vi "Global_SKM.vi"() -> ()   [LabVIEW 2025]
uses:
  Working condition setting_SKM.ctl
  data structure.ctl
panel:
  out "Stop":bool
  out "Wet Temp/RH":string[](array[string])
  in  "Information":string[][](array[string])=[["Date & Time", "02/23/2023 15:53:17"], ["Equipment Type Tested", "Chiller"], ["Refrigerant Type", ""], ["Operator Name", "qwe"], ["Test Duration (Time started/finished)", "fgh"], ["Job Reference Number", "120-20230209-01"], ["Unit Serial Number/EPN/SO Number", ""], ["Power Supply", ""], ["IPLV", ""], ["Test Report Number", ""], ["Refrigerant Charge", ""], ["Manufacturer/Brand Name", ""], ["Model Name/Series", ""], ["Test Standard", ""], ["Evaporator Type", ""], ["Evaporator Configuration", ""], ["Qty of Evaporator", ""], ["Evaporator 1 Model", ""], ["Evaporator 2 Model", ""], ["Evaporator 1 Serial #", ""], ["Evaporator 2 Serial #", ""], ["Condenser Type", ""], ["Qty of Condenser", ""], ["Number of Fans", ""], ["Number of actual running fans", ""], ["Rated Fan Speed", ""], ["Average Actual Fan Speed", ""], ["Rated Fan Motor Ampere", ""], ["Average Actual Fan Motor Ampere", ""], ["Qty of Compressor/Ckt", ""], ["Compressor Type", ""], ["Compressor Model", ""], ["Compressor Serial Number", ""], ["Refrigerant Charge", ""], ["Compressor Rated Load Amps", ""], ["Compressor Actual Ampere Drawn", ""], ["Compressor Type_Ckt2", ""], ["Compressor Model_Ckt2", ""], ["Compressor Serial Number_Ckt2", ""], ["Refrigerant Charge_Ckt2", ""], ["Compressor Rated Load Amps_Ckt2", ""], ["Compressor Actual Ampere Drawn_Ckt2", ""], ["Compressor Type_Ckt3", ""], ["Compressor Model_Ckt3", ""], ["Compressor Serial Number_Ckt3", ""], ["Refrigerant Charge_Ckt3", ""], ["Compressor Rated Load Amps_Ckt3", ""], ["Compressor Actual Ampere Drawn_Ckt3", ""], ["Compressor Type_Ckt4", ""], ["Compressor Model_Ckt4", ""], ["Compressor Serial Number_Ckt4", ""], ["Refrigerant Charge_Ckt4", ""], ["Compressor Rated Load Amps_Ckt4", ""], ["Compressor Actual Ampere Drawn_Ckt4", ""], ["Compressor Type_Ckt5", ""], ["Compressor Model_Ckt5", ""], ["Compressor Serial Number_Ckt5", ""], ["Refrigerant Charge_Ckt5", ""], ["Compressor Rated Load Amps_Ckt5", ""], ["Compressor Actual Ampere Drawn_Ckt5", ""], ["Compressor Type_Ckt6", ""], ["Compressor Model_Ckt6", ""], ["Compressor Serial Number_Ckt6", ""], ["Refrigerant Charge_Ckt6", ""], ["Compressor Rated Load Amps_Ckt6", ""], ["Compressor Actual Ampere Drawn_Ckt6", ""], ["Compressor Type_Ckt7", ""], ["Compressor Model_Ckt7", ""], ["Compressor Serial Number_Ckt7", ""], ["Refrigerant Charge_Ckt7", ""], ["Compressor Rated Load Amps_Ckt7", ""], ["Compressor Actual Ampere Drawn_Ckt7", ""], ["Compressor Type_Ckt8", ""], ["Compressor Model_Ckt8", ""], ["Compressor Serial Number_Ckt8", ""], ["Refrigerant Charge_Ckt8", ""], ["Compressor Rated Load Amps_Ckt8", ""], ["Compressor Actual Ampere Drawn_Ckt8", ""], ["Exp Valve Opening_Ckt1 ", ""], ["Exp Valve Opening_Ckt2", ""], ["Exp Valve Opening_Ckt3", ""], ["Exp Valve Opening_Ckt4", ""], ["Exp Valve Opening_Ckt5", ""], ["Exp Valve Opening_Ckt6", ""], ["Exp Valve Opening_Ckt7", ""], ["Exp Valve Opening_Ckt8", ""]]
  out "simu":bool
  in  "Correction_Data":dbl[][][](array[numeric])
  in  "数据结构组":T1[](array[typedef])=[{"展示名称"="U1_1", "单位"="V", "值"="", "物理通道"=240, "逻辑通道"=0, "小数点"=2, "数值"=0.0, "修正因子"={"a"=0.0, "b"=1.0, "c"=0.0}, "原始值"=0.0, "逻辑名称"="U1_1"}, {"展示名称"="I1_1", "单位"="A", "值"="", "物理通道"=241, "逻辑通道"=1, "小数点"=2, "数值"=0.0, "修正因子"={"a"=0.0, "b"=1.0, "c"=0.0}, "原始值"=0.0, "逻辑名称"="I1_1"}, {"展示名称"="P1_1", "单位"="W", "值"="", "物理通道"=242, "逻辑通道"=2, "小数点"=2, "数值"=0.0, "修正因子"={"a"=0.0, "b"=1.0, "c"=0.0}, "原始值"=0.0, "逻辑名称"="P1_1"}, {"展示名称"="E1_1", "单位"="W·h", "值"="", "物理通道"=243, "逻辑通道"=3, "小数点"=2, "数值"=0.0, "修正因子"={"a"=0.0, "b"=1.0, "c"=0.0}, "原始值"=0.0, "逻辑名称"="E1_1"}, {"展示名称"="U1_2", "单位"="V", "值"="", "物理通道"=244, "逻辑通道"=4, "小数点"=2, "数值"=0.0, "修正因子"={"a"=0.0, "b"=1.0, "c"=0.0}, "原始值"=0.0, "逻辑名称"="U1_2"}, {"展示名称"="I1_2", "单位"="A", "值"="", "物理通道"=245, "逻辑通道"=5, "小数点"=2, "数值"=0.0, "修正因子"={"a"=0.0, "b"=1.0, "c"=0.0}, "原始值"=0.0, "逻辑名称"="I1_2"}, {"展示名称"="P1_2", "单位"="W", "值"="", "物理通道"=246, "逻辑通道"=6, "小数点"=2, "数值"=0.0, "修正因子"={"a"=0.0, "b"=1.0, "c"=0.0}, "原始值"=0.0, "逻辑名称"="P1_2"}, {"展示名称"="E1_2", "单位"="W·h", "值"="", "物理通道"=247, "逻辑通道"=7, "小数点"=2, "数值"=0.0, "修正因子"={"a"=0.0, "b"=1.0, "c"=0.0}, "原始值"=0.0, "逻辑名称"="E1_2"}, {"展示名称"="U1_3", "单位"="V", "值"="", "物理通道"=248, "逻辑通道"=8, "小数点"=2, "数值"=0.0, "修正因子"={"a"=0.0, "b"=1.0, "c"=0.0}, "原始值"=0.0, "逻辑名称"="U1_3"}, {"展示名称"="I1_3", "单位"="A", "值"="", "物理通道"=249, "逻辑通道"=9, "小数点"=2, "数值"=0.0, "修正因子"={"a"=0.0, "b"=1.0, "c"=0.0}, "原始值"=0.0, "逻辑名称"="I1_3"}, {"展示名称"="P1_3", "单位"="W", "值"="", "物理通道"=250, "逻辑通道"=10, "小数点"=2, "数值"=0.0, "修正因子"={"a"=0.0, "b"=1.0, "c"=0.0}, "原始值"=0.0, "逻辑名称"="P1_3"}, {"展示名称"="E1_3", "单位"="W·h", "值"="", "物理通道"=251, "逻辑通道"=11, "小数点"=2, "数值"=0.0, "修正因子"={"a"=0.0, "b"=1.0, "c"=0.0}, "原始值"=0.0, "逻辑名称"="E1_3"}, {"展示名称"="U1_4", "单位"="V", "值"="", "物理通道"=252, "逻辑通道"=12, "小数点"=2, "数值"=0.0, "修正因子"={"a"=0.0, "b"=1.0, "c"=0.0}, "原始值"=0.0, "逻辑名称"="U1_4"}, {"展示名称"="I1_4", "单位"="A", "值"="", "物理通道"=253, "逻辑通道"=13, "小数点"=2, "数值"=0.0, "修正因子"={"a"=0.0, "b"=1.0, "c"=0.0}, "原始值"=0.0, "逻辑名称"="I1_4"}, {"展示名称"="P1_4", "单位"="W", "值"="", "物理通道"=254, "逻辑通道"=14, "小数点"=3, "数值"=0.0, "修正因子"={"a"=0.0, "b"=1.0, "c"=0.0}, "原始值"=0.0, "逻辑名称"="P1_4"}, {"展示名称"="E1_4", "单位"="W·h", "值"="", "物理通道"=255, "逻辑通道"=15, "小数点"=3, "数值"=0.0, "修正因子"={"a"=0.0, "b"=1.0, "c"=0.0}, "原始值"=0.0, "逻辑名称"="E1_4"}, {"展示名称"="Fq1", "单位"="Hz", "值"="", "物理通道"=256, "逻辑通道"=16, "小数点"=3, "数值"=0.0, "修正因子"={"a"=0.0, "b"=1.0, "c"=0.0}, "原始值"=0.0, "逻辑名称"="Fq1"}, {"展示名称"="Factor1", "单位"="", "值"="", "物理通道"=257, "逻辑通道"=17, "小数点"=3, "数值"=0.0, "修正因子"={"a"=0.0, "b"=1.0, "c"=0.0}, "原始值"=0.0, "逻辑名称"="Factor1"}, {"展示名称"="U2_1", "单位"="V", "值"="", "物理通道"=260, "逻辑通道"=18, "小数点"=1, "数值"=0.0, "修正因子"={"a"=0.0, "b"=1.0, "c"=0.0}, "原始值"=0.0, "逻辑名称"="U2_1"}, {"展示名称"="I2_1", "单位"="A", "值"="", "物理通道"=261, "逻辑通道"=19, "小数点"=1, "数值"=0.0, "修正因子"={"a"=0.0, "b"=1.0, "c"=0.0}, "原始值"=0.0, "逻辑名称"="I2_1"}, {"展示名称"="P2_1", "单位"="W", "值"="", "物理通道"=262, "逻辑通道"=20, "小数点"=1, "数值"=0.0, "修正因子"={"a"=0.0, "b"=1.0, "c"=0.0}, "原始值"=0.0, "逻辑名称"="P2_1"}, {"展示名称"="E2_1", "单位"="W·h", "值"="", "物理通道"=263, "逻辑通道"=21, "小数点"=2, "数值"=0.0, "修正因子"={"a"=0.0, "b"=1.0, "c"=0.0}, "原始值"=0.0, "逻辑名称"="E2_1"}, {"展示名称"="U2_2", "单位"="V", "值"="", "物理通道"=264, "逻辑通道"=22, "小数点"=2, "数值"=0.0, "修正因子"={"a"=0.0, "b"=1.0, "c"=0.0}, "原始值"=0.0, "逻辑名称"="U2_2"}, {"展示名称"="I2_2", "单位"="A", "值"="", "物理通道"=265, "逻辑通道"=23, "小数点"=2, "数值"=0.0, "修正因子"={"a"=0.0, "b"=1.0, "c"=0.0}, "原始值"=0.0, "逻辑名称"="I2_2"}, {"展示名称"="P2_2", "单位"="W", "值"="", "物理通道"=266, "逻辑通道"=24, "小数点"=2, "数值"=0.0, "修正因子"={"a"=0.0, "b"=1.0, "c"=0.0}, "原始值"=0.0, "逻辑名称"="P2_2"}, {"展示名称"="E2_2", "单位"="W·h", "值"="", "物理通道"=267, "逻辑通道"=25, "小数点"=1, "数值"=0.0, "修正因子"={"a"=0.0, "b"=1.0, "c"=0.0}, "原始值"=0.0, "逻辑名称"="E2_2"}, {"展示名称"="U2_3", "单位"="V", "值"="", "物理通道"=268, "逻辑通道"=26, "小数点"=1, "数值"=0.0, "修正因子"={"a"=0.0, "b"=1.0, "c"=0.0}, "原始值"=0.0, "逻辑名称"="U2_3"}, {"展示名称"="I2_3", "单位"="A", "值"="", "物理通道"=269, "逻辑通道"=27, "小数点"=1, "数值"=0.0, "修正因子"={"a"=0.0, "b"=1.0, "c"=0.0}, "原始值"=0.0, "逻辑名称"="I2_3"}, {"展示名称"="P2_3", "单位"="W", "值"="", "物理通道"=270, "逻辑通道"=28, "小数点"=1, "数值"=0.0, "修正因子"={"a"=0.0, "b"=1.0, "c"=0.0}, "原始值"=0.0, "逻辑名称"="P2_3"}, {"展示名称"="E2_3", "单位"="W·h", "值"="", "物理通道"=271, "逻辑通道"=29, "小数点"=1, "数值"=0.0, "修正因子"={"a"=0.0, "b"=1.0, "c"=0.0}, "原始值"=0.0, "逻辑名称"="E2_3"}, {"展示名称"="U2_4", "单位"="V", "值"="", "物理通道"=272, "逻辑通道"=30, "小数点"=1, "数值"=0.0, "修正因子"={"a"=0.0, "b"=1.0, "c"=0.0}, "原始值"=0.0, "逻辑名称"="U2_4"}, {"展示名称"="I2_4", "单位"="A", "值"="", "物理通道"=273, "逻辑通道"=31, "小数点"=1, "数值"=0.0, "修正因子"={"a"=0.0, "b"=1.0, "c"=0.0}, "原始值"=0.0, "逻辑名称"="I2_4"}, {"展示名称"="P2_4", "单位"="W", "值"="", "物理通道"=274, "逻辑通道"=32, "小数点"=1, "数值"=0.0, "修正因子"={"a"=0.0, "b"=1.0, "c"=0.0}, "原始值"=0.0, "逻辑名称"="P2_4"}, {"展示名称"="E2_4", "单位"="W·h", "值"="", "物理通道"=275, "逻辑通道"=33, "小数点"=1, "数值"=0.0, "修正因子"={"a"=0.0, "b"=1.0, "c"=0.0}, "原始值"=0.0, "逻辑名称"="E2_4"}, {"展示名称"="Fq2", "单位"="Hz", "值"="", "物理通道"=276, "逻辑通道"=34, "小数点"=1, "数值"=0.0, "修正因子"={"a"=0.0, "b"=1.0, "c"=0.0}, "原始值"=0.0, "逻辑名称"="Fq2"}, {"展示名称"="Factor2", "单位"="", "值"="", "物理通道"=277, "逻辑通道"=35, "小数点"=1, "数值"=0.0, "修正因子"={"a"=0.0, "b"=1.0, "c"=0.0}, "原始值"=0.0, "逻辑名称"="Factor2"}, {"展示名称"="U3_1", "单位"="V", "值"="", "物理通道"=280, "逻辑通道"=36, "小数点"=1, "数值"=0.0, "修正因子"={"a"=0.0, "b"=1.0, "c"=0.0}, "原始值"=0.0, "逻辑名称"="U3_1"}, {"展示名称"="I3_1", "单位"="A", "值"="", "物理通道"=281, "逻辑通道"=37, "小数点"=1, "数值"=0.0, "修正因子"={"a"=0.0, "b"=1.0, "c"=0.0}, "原始值"=0.0, "逻辑名称"="I3_1"}, {"展示名称"="P3_1", "单位"="W", "值"="", "物理通道"=282, "逻辑通道"=38, "小数点"=1, "数值"=0.0, "修正因子"={"a"=0.0, "b"=1.0, "c"=0.0}, "原始值"=0.0, "逻辑名称"="P3_1"}, {"展示名称"="E3_1", "单位"="W·h", "值"="", "物理通道"=283, "逻辑通道"=39, "小数点"=1, "数值"=0.0, "修正因子"={"a"=0.0, "b"=1.0, "c"=0.0}, "原始值"=0.0, "逻辑名称"="E3_1"}, {"展示名称"="U3_2", "单位"="V", "值"="", "物理通道"=284, "逻辑通道"=40, "小数点"=1, "数值"=0.0, "修正因子"={"a"=0.0, "b"=1.0, "c"=0.0}, "原始值"=0.0, "逻辑名称"="U3_2"}, {"展示名称"="I3_2", "单位"="A", "值"="", "物理通道"=285, "逻辑通道"=41, "小数点"=1, "数值"=0.0, "修正因子"={"a"=0.0, "b"=1.0, "c"=0.0}, "原始值"=0.0, "逻辑名称"="I3_2"}, {"展示名称"="P3_2", "单位"="W", "值"="", "物理通道"=286, "逻辑通道"=42, "小数点"=1, "数值"=0.0, "修正因子"={"a"=0.0, "b"=1.0, "c"=0.0}, "原始值"=0.0, "逻辑名称"="P3_2"}, {"展示名称"="E3_2", "单位"="W·h", "值"="", "物理通道"=287, "逻辑通道"=43, "小数点"=1, "数值"=0.0, "修正因子"={"a"=0.0, "b"=1.0, "c"=0.0}, "原始值"=0.0, "逻辑名称"="E3_2"}, {"展示名称"="U3_3", "单位"="V", "值"="", "物理通道"=288, "逻辑通道"=44, "小数点"=1, "数值"=0.0, "修正因子"={"a"=0.0, "b"=1.0, "c"=0.0}, "原始值"=0.0, "逻辑名称"="U3_3"}, {"展示名称"="I3_3", "单位"="A", "值"="", "物理通道"=289, "逻辑通道"=45, "小数点"=1, "数值"=0.0, "修正因子"={"a"=0.0, "b"=1.0, "c"=0.0}, "原始值"=0.0, "逻辑名称"="I3_3"}, {"展示名称"="P3_3", "单位"="W", "值"="", "物理通道"=290, "逻辑通道"=46, "小数点"=1, "数值"=0.0, "修正因子"={"a"=0.0, "b"=1.0, "c"=0.0}, "原始值"=0.0, "逻辑名称"="P3_3"}, {"展示名称"="E3_3", "单位"="W·h", "值"="", "物理通道"=291, "逻辑通道"=47, "小数点"=1, "数值"=0.0, "修正因子"={"a"=0.0, "b"=1.0, "c"=0.0}, "原始值"=0.0, "逻辑名称"="E3_3"}, {"展示名称"="U3_4", "单位"="V", "值"="", "物理通道"=292, "逻辑通道"=48, "小数点"=1, "数值"=0.0, "修正因子"={"a"=0.0, "b"=1.0, "c"=0.0}, "原始值"=0.0, "逻辑名称"="U3_4"}, {"展示名称"="I3_4", "单位"="A", "值"="", "物理通道"=293, "逻辑通道"=49, "小数点"=1, "数值"=0.0, "修正因子"={"a"=0.0, "b"=1.0, "c"=0.0}, "原始值"=0.0, "逻辑名称"="I3_4"}, {"展示名称"="P3_4", "单位"="W", "值"="", "物理通道"=294, "逻辑通道"=50, "小数点"=1, "数值"=0.0, "修正因子"={"a"=0.0, "b"=1.0, "c"=0.0}, "原始值"=0.0, "逻辑名称"="P3_4"}, {"展示名称"="E3_4", "单位"="W·h", "值"="", "物理通道"=295, "逻辑通道"=51, "小数点"=1, "数值"=0.0, "修正因子"={"a"=0.0, "b"=1.0, "c"=0.0}, "原始值"=0.0, "逻辑名称"="E3_4"}, {"展示名称"="Fq3", "单位"="Hz", "值"="", "物理通道"=296, "逻辑通道"=52, "小数点"=1, "数值"=0.0, "修正因子"={"a"=0.0, "b"=1.0, "c"=0.0}, "原始值"=0.0, "逻辑名称"="Fq3"}, {"展示名称"="Factor3", "单位"="", "值"="", "物理通道"=297, "逻辑通道"=53, "小数点"=1, "数值"=0.0, "修正因子"={"a"=0.0, "b"=1.0, "c"=0.0}, "原始值"=0.0, "逻辑名称"="Factor3"}, {"展示名称"="U4_1", "单位"="V", "值"="", "物理通道"=300, "逻辑通道"=54, "小数点"=1, "数值"=0.0, "修正因子"={"a"=0.0, "b"=1.0, "c"=0.0}, "原始值"=0.0, "逻辑名称"="U4_1"}, {"展示名称"="I4_1", "单位"="A", "值"="", "物理通道"=301, "逻辑通道"=55, "小数点"=1, "数值"=0.0, "修正因子"={"a"=0.0, "b"=1.0, "c"=0.0}, "原始值"=0.0, "逻辑名称"="I4_1"}, {"展示名称"="P4_1", "单位"="W", "值"="", "物理通道"=302, "逻辑通道"=56, "小数点"=1, "数值"=0.0, "修正因子"={"a"=0.0, "b"=1.0, "c"=0.0}, "原始值"=0.0, "逻辑名称"="P4_1"}, {"展示名称"="E4_1", "单位"="W·h", "值"="", "物理通道"=303, "逻辑通道"=57, "小数点"=1, "数值"=0.0, "修正因子"={"a"=0.0, "b"=1.0, "c"=0.0}, "原始值"=0.0, "逻辑名称"="E4_1"}, {"展示名称"="U4_2", "单位"="V", "值"="", "物理通道"=304, "逻辑通道"=58, "小数点"=1, "数值"=0.0, "修正因子"={"a"=0.0, "b"=1.0, "c"=0.0}, "原始值"=0.0, "逻辑名称"="U4_2"}, {"展示名称"="I4_2", "单位"="A", "值"="", "物理通道"=305, "逻辑通道"=59, "小数点"=1, "数值"=0.0, "修正因子"={"a"=0.0, "b"=1.0, "c"=0.0}, "原始值"=0.0, "逻辑名称"="I4_2"}, {"展示名称"="P4_2", "单位"="W", "值"="", "物理通道"=306, "逻辑通道"=60, "小数点"=1, "数值"=0.0, "修正因子"={"a"=0.0, "b"=1.0, "c"=0.0}, "原始值"=0.0, "逻辑名称"="P4_2"}, {"展示名称"="E4_2", "单位"="W·h", "值"="", "物理通道"=307, "逻辑通道"=61, "小数点"=1, "数值"=0.0, "修正因子"={"a"=0.0, "b"=1.0, "c"=0.0}, "原始值"=0.0, "逻辑名称"="E4_2"}, {"展示名称"="U4_3", "单位"="V", "值"="", "物理通道"=308, "逻辑通道"=62, "小数点"=1, "数值"=0.0, "修正因子"={"a"=0.0, "b"=1.0, "c"=0.0}, "原始值"=0.0, "逻辑名称"="U4_3"}, {"展示名称"="I4_3", "单位"="A", "值"="", "物理通道"=309, "逻辑通道"=63, "小数点"=1, "数值"=0.0, "修正因子"={"a"=0.0, "b"=1.0, "c"=0.0}, "原始值"=0.0, "逻辑名称"="I4_3"}, {"展示名称"="P4_3", "单位"="W", "值"="", "物理通道"=310, "逻辑通道"=64, "小数点"=1, "数值"=0.0, "修正因子"={"a"=0.0, "b"=1.0, "c"=0.0}, "原始值"=0.0, "逻辑名称"="P4_3"}, {"展示名称"="E4_3", "单位"="W·h", "值"="", "物理通道"=311, "逻辑通道"=65, "小数点"=1, "数值"=0.0, "修正因子"={"a"=0.0, "b"=1.0, "c"=0.0}, "原始值"=0.0, "逻辑名称"="E4_3"}, {"展示名称"="U4_4", "单位"="V", "值"="", "物理通道"=312, "逻辑通道"=66, "小数点"=1, "数值"=0.0, "修正因子"={"a"=0.0, "b"=1.0, "c"=0.0}, "原始值"=0.0, "逻辑名称"="U4_4"}, {"展示名称"="I4_4", "单位"="A", "值"="", "物理通道"=313, "逻辑通道"=67, "小数点"=1, "数值"=0.0, "修正因子"={"a"=0.0, "b"=1.0, "c"=0.0}, "原始值"=0.0, "逻辑名称"="I4_4"}, {"展示名称"="P4_4", "单位"="W", "值"="", "物理通道"=314, "逻辑通道"=68, "小数点"=1, "数值"=0.0, "修正因子"={"a"=0.0, "b"=1.0, "c"=0.0}, "原始值"=0.0, "逻辑名称"="P4_4"}, {"展示名称"="E4_4", "单位"="W·h", "值"="", "物理通道"=315, "逻辑通道"=69, "小数点"=1, "数值"=0.0, "修正因子"={"a"=0.0, "b"=1.0, "c"=0.0}, "原始值"=0.0, "逻辑名称"="E4_4"}, {"展示名称"="Fq4", "单位"="Hz", "值"="", "物理通道"=316, "逻辑通道"=70, "小数点"=1, "数值"=0.0, "修正因子"={"a"=0.0, "b"=1.0, "c"=0.0}, "原始值"=0.0, "逻辑名称"="Fq4"}, {"展示名称"="Factor4", "单位"="", "值"="", "物理通道"=317, "逻辑通道"=71, "小数点"=1, "数值"=0.0, "修正因子"={"a"=0.0, "b"=1.0, "c"=0.0}, "原始值"=0.0, "逻辑名称"="Factor4"}, {"展示名称"="U5_1", "单位"="V", "值"="", "物理通道"=320, "逻辑通道"=72, "小数点"=1, "数值"=0.0, "修正因子"={"a"=0.0, "b"=1.0, "c"=0.0}, "原始值"=0.0, "逻辑名称"="U5_1"}, {"展示名称"="I5_1", "单位"="A", "值"="", "物理通道"=321, "逻辑通道"=73, "小数点"=1, "数值"=0.0, "修正因子"={"a"=0.0, "b"=1.0, "c"=0.0}, "原始值"=0.0, "逻辑名称"="I5_1"}, {"展示名称"="P5_1", "单位"="W", "值"="", "物理通道"=322, "逻辑通道"=74, "小数点"=1, "数值"=0.0, "修正因子"={"a"=0.0, "b"=1.0, "c"=0.0}, "原始值"=0.0, "逻辑名称"="P5_1"}, {"展示名称"="E5_1", "单位"="W·h", "值"="", "物理通道"=323, "逻辑通道"=75, "小数点"=1, "数值"=0.0, "修正因子"={"a"=0.0, "b"=1.0, "c"=0.0}, "原始值"=0.0, "逻辑名称"="E5_1"}, {"展示名称"="U5_2", "单位"="V", "值"="", "物理通道"=324, "逻辑通道"=76, "小数点"=1, "数值"=0.0, "修正因子"={"a"=0.0, "b"=1.0, "c"=0.0}, "原始值"=0.0, "逻辑名称"="U5_2"}, {"展示名称"="I5_2", "单位"="A", "值"="", "物理通道"=325, "逻辑通道"=77, "小数点"=1, "数值"=0.0, "修正因子"={"a"=0.0, "b"=1.0, "c"=0.0}, "原始值"=0.0, "逻辑名称"="I5_2"}, {"展示名称"="P5_2", "单位"="W", "值"="", "物理通道"=326, "逻辑通道"=78, "小数点"=1, "数值"=0.0, "修正因子"={"a"=0.0, "b"=1.0, "c"=0.0}, "原始值"=0.0, "逻辑名称"="P5_2"}, {"展示名称"="E5_2", "单位"="W·h", "值"="", "物理通道"=327, "逻辑通道"=79, "小数点"=1, "数值"=0.0, "修正因子"={"a"=0.0, "b"=1.0, "c"=0.0}, "原始值"=0.0, "逻辑名称"="E5_2"}, {"展示名称"="U5_3", "单位"="V", "值"="", "物理通道"=328, "逻辑通道"=80, "小数点"=1, "数值"=0.0, "修正因子"={"a"=0.0, "b"=1.0, "c"=0.0}, "原始值"=0.0, "逻辑名称"="U5_3"}, {"展示名称"="I5_3", "单位"="A", "值"="", "物理通道"=329, "逻辑通道"=81, "小数点"=1, "数值"=0.0, "修正因子"={"a"=0.0, "b"=1.0, "c"=0.0}, "原始值"=0.0, "逻辑名称"="I5_3"}, {"展示名称"="P5_3", "单位"="W", "值"="", "物理通道"=330, "逻辑通道"=82, "小数点"=1, "数值"=0.0, "修正因子"={"a"=0.0, "b"=1.0, "c"=0.0}, "原始值"=0.0, "逻辑名称"="P5_3"}, {"展示名称"="E5_3", "单位"="W·h", "值"="", "物理通道"=331, "逻辑通道"=83, "小数点"=1, "数值"=0.0, "修正因子"={"a"=0.0, "b"=1.0, "c"=0.0}, "原始值"=0.0, "逻辑名称"="E5_3"}, {"展示名称"="U5_4", "单位"="V", "值"="", "物理通道"=332, "逻辑通道"=84, "小数点"=1, "数值"=0.0, "修正因子"={"a"=0.0, "b"=1.0, "c"=0.0}, "原始值"=0.0, "逻辑名称"="U5_4"}, {"展示名称"="I5_4", "单位"="A", "值"="", "物理通道"=333, "逻辑通道"=85, "小数点"=1, "数值"=0.0, "修正因子"={"a"=0.0, "b"=1.0, "c"=0.0}, "原始值"=0.0, "逻辑名称"="I5_4"}, {"展示名称"="P5_4", "单位"="W", "值"="", "物理通道"=334, "逻辑通道"=86, "小数点"=1, "数值"=0.0, "修正因子"={"a"=0.0, "b"=1.0, "c"=0.0}, "原始值"=0.0, "逻辑名称"="P5_4"}, {"展示名称"="E5_4", "单位"="W·h", "值"="", "物理通道"=335, "逻辑通道"=87, "小数点"=1, "数值"=0.0, "修正因子"={"a"=0.0, "b"=1.0, "c"=0.0}, "原始值"=0.0, "逻辑名称"="E5_4"}, {"展示名称"="Fq5", "单位"="Hz", "值"="", "物理通道"=336, "逻辑通道"=88, "小数点"=1, "数值"=0.0, "修正因子"={"a"=0.0, "b"=1.0, "c"=0.0}, "原始值"=0.0, "逻辑名称"="Fq5"}, {"展示名称"="Factor5", "单位"="", "值"="", "物理通道"=337, "逻辑通道"=89, "小数点"=1, "数值"=0.0, "修正因子"={"a"=0.0, "b"=1.0, "c"=0.0}, "原始值"=0.0, "逻辑名称"="Factor5"}, {"展示名称"="25TR SAMLL CHAMBER AC OUTLET DRY_BULB TEMP.", "单位"="℃", "值"="", "物理通道"=340, "逻辑通道"=90, "小数点"=1, "数值"=0.0, "修正因子"={"a"=0.0, "b"=1.0, "c"=0.0}, "原始值"=0.0, "逻辑名称"="25TR SAMLL CHAMBER AC OUTLET DRY_BULB TEMP."}, {"展示名称"="25TR SMALL CHAMBER AC OUTLET WET_BULB TEMP.", "单位"="℃", "值"="", "物理通道"=341, "逻辑通道"=91, "小数点"=1, "数值"=0.0, "修正因子"={"a"=0.0, "b"=1.0, "c"=0.0}, "原始值"=0.0, "逻辑名称"="25TR SMALL CHAMBER AC OUTLET WET_BULB TEMP."}, {"展示名称"="25TR SMALL CHAMBER BEF. NOZZLE DRY_BULB TEMP.", "单位"="℃", "值"="", "物理通道"=342, "逻辑通道"=92, "小数点"=1, "数值"=0.0, "修正因子"={"a"=0.0, "b"=1.0, "c"=0.0}, "原始值"=0.0, "逻辑名称"="25TR SMALL CHAMBER BEF. NOZZLE DRY_BULB TEMP."}, {"展示名称"="25TR BIG CHAMBER AC OUTLET DRY_BULB TEMP.", "单位"="℃", "值"="", "物理通道"=343, "逻辑通道"=93, "小数点"=1, "数值"=0.0, "修正因子"={"a"=0.0, "b"=1.0, "c"=0.0}, "原始值"=0.0, "逻辑名称"="25TR BIG CHAMBER AC OUTLET DRY_BULB TEMP."}, {"展示名称"="25TR BIG CHAMBER AC OUTLET WET_BULB TEMP.", "单位"="℃", "值"="", "物理通道"=344, "逻辑通道"=94, "小数点"=1, "数值"=0.0, "修正因子"={"a"=0.0, "b"=1.0, "c"=0.0}, "原始值"=0.0, "逻辑名称"="25TR BIG CHAMBER AC OUTLET WET_BULB TEMP."}, {"展示名称"="25TR BIG CHAMBER BEF. NOZZLE DRY_BULB TEMP.", "单位"="℃", "值"="", "物理通道"=345, "逻辑通道"=95, "小数点"=1, "数值"=0.0, "修正因子"={"a"=0.0, "b"=1.0, "c"=0.0}, "原始值"=0.0, "逻辑名称"="25TR BIG CHAMBER BEF. NOZZLE DRY_BULB TEMP."}, {"展示名称"="50TR SAMLL CHAMBER AC OUTLET DRY_BULB TEMP.", "单位"="℃", "值"="", "物理通道"=346, "逻辑通道"=96, "小数点"=1, "数值"=0.0, "修正因子"={"a"=0.0, "b"=1.0, "c"=0.0}, "原始值"=0.0, "逻辑名称"="50TR SAMLL CHAMBER AC OUTLET DRY_BULB TEMP."}, {"展示名称"="50TR SMALL CHAMBER AC OUTLET WET_BULB TEMP.", "单位"="℃", "值"="", "物理通道"=347, "逻辑通道"=97, "小数点"=1, "数值"=0.0, "修正因子"={"a"=0.0, "b"=1.0, "c"=0.0}, "原始值"=0.0, "逻辑名称"="50TR SMALL CHAMBER AC OUTLET WET_BULB TEMP."}, {"展示名称"="50TR SMALL CHAMBER BEF. NOZZLE DRY_BULB TEMP.", "单位"="℃", "值"="", "物理通道"=348, "逻辑通道"=98, "小数点"=1, "数值"=0.0, "修正因子"={"a"=0.0, "b"=1.0, "c"=0.0}, "原始值"=0.0, "逻辑名称"="50TR SMALL CHAMBER BEF. NOZZLE DRY_BULB TEMP."}, {"展示名称"="50TR BIG CHAMBER AC OUTLET DRY_BULB TEMP.", "单位"="℃", "值"="", "物理通道"=349, "逻辑通道"=99, "小数点"=1, "数值"=0.0, "修正因子"={"a"=0.0, "b"=1.0, "c"=0.0}, "原始值"=0.0, "逻辑名称"="50TR BIG CHAMBER AC OUTLET DRY_BULB TEMP."}, {"展示名称"="50TR BIG CHAMBER AC OUTLET WET_BULB TEMP.", "单位"="℃", "值"="", "物理通道"=362, "逻辑通道"=100, "小数点"=1, "数值"=0.0, "修正因子"={"a"=0.0, "b"=1.0, "c"=0.0}, "原始值"=0.0, "逻辑名称"="50TR BIG CHAMBER AC OUTLET WET_BULB TEMP."}, {"展示名称"="50TR BIG CHAMBER BEF. NOZZLE DRY_BULB TEMP.", "单位"="℃", "值"="", "物理通道"=363, "逻辑通道"=101, "小数点"=1, "数值"=0.0, "修正因子"={"a"=0.0, "b"=1.0, "c"=0.0}, "原始值"=0.0, "逻辑名称"="50TR BIG CHAMBER BEF. NOZZLE DRY_BULB TEMP."}, {"展示名称"="25TR WATER SYSTEM INLET TEMP.", "单位"="℃", "值"="", "物理通道"=364, "逻辑通道"=102, "小数点"=1, "数值"=0.0, "修正因子"={"a"=0.0, "b"=1.0, "c"=0.0}, "原始值"=0.0, "逻辑名称"="25TR WATER SYSTEM INLET TEMP."}, {"展示名称"="25TR WATER SYSTEM OUTLET TEMP.", "单位"="℃", "值"="", "物理通道"=365, "逻辑通道"=103, "小数点"=1, "数值"=0.0, "修正因子"={"a"=0.0, "b"=1.0, "c"=0.0}, "原始值"=0.0, "逻辑名称"="25TR WATER SYSTEM OUTLET TEMP."}, {"展示名称"="50TR WATER SYSTEM INTLET TEMP.", "单位"="℃", "值"="", "物理通道"=366, "逻辑通道"=104, "小数点"=1, "数值"=0.0, "修正因子"={"a"=0.0, "b"=1.0, "c"=0.0}, "原始值"=0.0, "逻辑名称"="50TR WATER SYSTEM INTLET TEMP."}, {"展示名称"="50TR WATER SYSTEM OUTLET TEMP.", "单位"="℃", "值"="", "物理通道"=367, "逻辑通道"=105, "小数点"=1, "数值"=0.0, "修正因子"={"a"=0.0, "b"=1.0, "c"=0.0}, "原始值"=0.0, "逻辑名称"="50TR WATER SYSTEM OUTLET TEMP."}, {"展示名称"="PT117", "单位"="℃", "值"="", "物理通道"=367, "逻辑通道"=106, "小数点"=1, "数值"=0.0, "修正因子"={"a"=0.0, "b"=1.0, "c"=0.0}, "原始值"=0.0, "逻辑名称"="Ref.TEMP.-1"}, {"展示名称"="PT118", "单位"="℃", "值"="", "物理通道"=367, "逻辑通道"=107, "小数点"=1, "数值"=0.0, "修正因子"={"a"=0.0, "b"=1.0, "c"=0.0}, "原始值"=0.0, "逻辑名称"="Ref.TEMP.-2"}, {"展示名称"="PT119", "单位"="℃", "值"="", "物理通道"=367, "逻辑通道"=108, "小数点"=1, "数值"=0.0, "修正因子"={"a"=0.0, "b"=1.0, "c"=0.0}, "原始值"=0.0, "逻辑名称"="Ref.TEMP.-3"}, {"展示名称"="PT120", "单位"="℃", "值"="", "物理通道"=367, "逻辑通道"=109, "小数点"=1, "数值"=0.0, "修正因子"={"a"=0.0, "b"=1.0, "c"=0.0}, "原始值"=0.0, "逻辑名称"="Ref.TEMP.-4"}, {"展示名称"="PT121", "单位"="℃", "值"="", "物理通道"=384, "逻辑通道"=110, "小数点"=1, "数值"=0.0, "修正因子"={"a"=0.0, "b"=1.0, "c"=0.0}, "原始值"=0.0, "逻辑名称"="Ref.TEMP.-5"}, {"展示名称"="PT122", "单位"="℃", "值"="", "物理通道"=385, "逻辑通道"=111, "小数点"=1, "数值"=0.0, "修正因子"={"a"=0.0, "b"=1.0, "c"=0.0}, "原始值"=0.0, "逻辑名称"="Ref.TEMP.-6"}, {"展示名称"="PT123", "单位"="℃", "值"="", "物理通道"=386, "逻辑通道"=112, "小数点"=1, "数值"=0.0, "修正因子"={"a"=0.0, "b"=1.0, "c"=0.0}, "原始值"=0.0, "逻辑名称"="Ref.TEMP.-7"}, {"展示名称"="PT124", "单位"="℃", "值"="", "物理通道"=387, "逻辑通道"=113, "小数点"=1, "数值"=0.0, "修正因子"={"a"=0.0, "b"=1.0, "c"=0.0}, "原始值"=0.0, "逻辑名称"="Ref.TEMP.-8"}, {"展示名称"="PT125", "单位"="℃", "值"="", "物理通道"=388, "逻辑通道"=114, "小数点"=1, "数值"=0.0, "修正因子"={"a"=0.0, "b"=1.0, "c"=0.0}, "原始值"=0.0, "逻辑名称"="Ref.TEMP.-9"}, {"展示名称"="PT126", "单位"="℃", "值"="", "物理通道"=389, "逻辑通道"=115, "小数点"=1, "数值"=0.0, "修正因子"={"a"=0.0, "b"=1.0, "c"=0.0}, "原始值"=0.0, "逻辑名称"="Ref.TEMP.-10"}, {"展示名称"="PT127", "单位"="℃", "值"="", "物理通道"=390, "逻辑通道"=116, "小数点"=1, "数值"=0.0, "修正因子"={"a"=0.0, "b"=1.0, "c"=0.0}, "原始值"=0.0, "逻辑名称"="Ref.TEMP.-11"}, {"展示名称"="PT128", "单位"="℃", "值"="", "物理通道"=391, "逻辑通道"=117, "小数点"=1, "数值"=0.0, "修正因子"={"a"=0.0, "b"=1.0, "c"=0.0}, "原始值"=0.0, "逻辑名称"="Ref.TEMP.-12"}, {"展示名称"="SP1", "单位"="Mpa", "值"="", "物理通道"=406, "逻辑通道"=118, "小数点"=1, "数值"=0.0, "修正因子"={"a"=0.0, "b"=1.0, "c"=0.0}, "原始值"=0.0, "逻辑名称"="Ref P1(SP1)"}, {"展示名称"="SP2", "单位"="Mpa", "值"="", "物理通道"=407, "逻辑通道"=119, "小数点"=1, "数值"=0.0, "修正因子"={"a"=0.0, "b"=1.0, "c"=0.0}, "原始值"=0.0, "逻辑名称"="Ref P2(SP2)"}, {"展示名称"="SP3", "单位"="Mpa", "值"="", "物理通道"=408, "逻辑通道"=120, "小数点"=1, "数值"=0.0, "修正因子"={"a"=0.0, "b"=1.0, "c"=0.0}, "原始值"=0.0, "逻辑名称"="Ref P3(SP3)"}, {"展示名称"="SP4", "单位"="Mpa", "值"="", "物理通道"=409, "逻辑通道"=121, "小数点"=1, "数值"=0.0, "修正因子"={"a"=0.0, "b"=1.0, "c"=0.0}, "原始值"=0.0, "逻辑名称"="Ref P4(SP4)"}, {"展示名称"="SP5", "单位"="Mpa", "值"="", "物理通道"=410, "逻辑通道"=122, "小数点"=1, "数值"=0.0, "修正因子"={"a"=0.0, "b"=1.0, "c"=0.0}, "原始值"=0.0, "逻辑名称"="Ref P5(SP5)"}, {"展示名称"="SP6", "单位"="Mpa", "值"="", "物理通道"=411, "逻辑通道"=123, "小数点"=1, "数值"=0.0, "修正因子"={"a"=0.0, "b"=1.0, "c"=0.0}, "原始值"=0.0, "逻辑名称"="Ref P6(SP6)"}, {"展示名称"="SP7", "单位"="Mpa", "值"="", "物理通道"=412, "逻辑通道"=124, "小数点"=1, "数值"=0.0, "修正因子"={"a"=0.0, "b"=1.0, "c"=0.0}, "原始值"=0.0, "逻辑名称"="Ref P7(SP7)"}, {"展示名称"="SP8", "单位"="Mpa", "值"="", "物理通道"=413, "逻辑通道"=125, "小数点"=1, "数值"=0.0, "修正因子"={"a"=0.0, "b"=1.0, "c"=0.0}, "原始值"=0.0, "逻辑名称"="Ref P8(SP8)"}, {"展示名称"="SP9", "单位"="Mpa", "值"="", "物理通道"=414, "逻辑通道"=126, "小数点"=1, "数值"=0.0, "修正因子"={"a"=0.0, "b"=1.0, "c"=0.0}, "原始值"=0.0, "逻辑名称"="Ref P9(SP9)"}, {"展示名称"="SP10", "单位"="Mpa", "值"="", "物理通道"=415, "逻辑通道"=127, "小数点"=1, "数值"=0.0, "修正因子"={"a"=0.0, "b"=1.0, "c"=0.0}, "原始值"=0.0, "逻辑名称"="Ref P10(SP10)"}, {"展示名称"="SP11", "单位"="Mpa", "值"="", "物理通道"=416, "逻辑通道"=128, "小数点"=1, "数值"=0.0, "修正因子"={"a"=0.0, "b"=1.0, "c"=0.0}, "原始值"=0.0, "逻辑名称"="Ref P11(SP11)"}, {"展示名称"="SP12", "单位"="Mpa", "值"="", "物理通道"=417, "逻辑通道"=129, "小数点"=1, "数值"=0.0, "修正因子"={"a"=0.0, "b"=1.0, "c"=0.0}, "原始值"=0.0, "逻辑名称"="Ref P12(SP12)"}, {"展示名称"="FM3", "单位"="m3/h", "值"="", "物理通道"=418, "逻辑通道"=130, "小数点"=1, "数值"=0.0, "修正因子"={"a"=0.0, "b"=1.0, "c"=0.0}, "原始值"=0.0, "逻辑名称"="Ref.Mass Flow Meter1"}, {"展示名称"="FM4", "单位"="m3/h", "值"="", "物理通道"=419, "逻辑通道"=131, "小数点"=1, "数值"=0.0, "修正因子"={"a"=0.0, "b"=1.0, "c"=0.0}, "原始值"=0.0, "逻辑名称"="Ref.Mass Flow Meter1"}, {"展示名称"="25TR Water System Test Unit Water Pressure", "单位"="Mpa", "值"="", "物理通道"=420, "逻辑通道"=132, "小数点"=1, "数值"=0.0, "修正因子"={"a"=0.0, "b"=1.0, "c"=0.0}, "原始值"=0.0, "逻辑名称"="25TR Water System Test Unit Water Pressure"}, {"展示名称"="50TR Water System Test Unit Water Pressure Difference(DP6)", "单位"="Mpa", "值"="", "物理通道"=421, "逻辑通道"=133, "小数点"=1, "数值"=0.0, "修正因子"={"a"=0.0, "b"=1.0, "c"=0.0}, "原始值"=0.0, "逻辑名称"="50TR Water System Test Unit Water Pressure Difference(DP6)"}, {"展示名称"="25TR Indoor room RH", "单位"="%", "值"="", "物理通道"=422, "逻辑通道"=134, "小数点"=1, "数值"=0.0, "修正因子"={"a"=0.0, "b"=1.0, "c"=0.0}, "原始值"=0.0, "逻辑名称"="25TR Indoor room RH"}, {"展示名称"="50TR Indoor room RH", "单位"="%", "值"="", "物理通道"=423, "逻辑通道"=135, "小数点"=1, "数值"=0.0, "修正因子"={"a"=0.0, "b"=1.0, "c"=0.0}, "原始值"=0.0, "逻辑名称"="50TR Indoor room RH"}, {"展示名称"="50TR Outdoor room RH1", "单位"="%", "值"="", "物理通道"=424, "逻辑通道"=136, "小数点"=1, "数值"=0.0, "修正因子"={"a"=0.0, "b"=1.0, "c"=0.0}, "原始值"=0.0, "逻辑名称"="50TR Outdoor room RH1"}, {"展示名称"="50TR Outdoor room RH2", "单位"="%", "值"="", "物理通道"=425, "逻辑通道"=137, "小数点"=1, "数值"=0.0, "修正因子"={"a"=0.0, "b"=1.0, "c"=0.0}, "原始值"=0.0, "逻辑名称"="50TR Outdoor room RH2"}, {"展示名称"="25TR Small Chamber Nozzle Pressure Difference", "单位"="Mpa", "值"="", "物理通道"=426, "逻辑通道"=138, "小数点"=1, "数值"=0.0, "修正因子"={"a"=0.0, "b"=1.0, "c"=0.0}, "原始值"=0.0, "逻辑名称"="25TR Small Chamber Nozzle Pressure Difference"}, {"展示名称"="25TR Big Chamber Nozzle Pressure Difference", "单位"="Mpa", "值"="", "物理通道"=427, "逻辑通道"=139, "小数点"=1, "数值"=0.0, "修正因子"={"a"=0.0, "b"=1.0, "c"=0.0}, "原始值"=0.0, "逻辑名称"="25TR Big Chamber Nozzle Pressure Difference"}, {"展示名称"="Barometric Pressure(DP7)", "单位"="Mpa", "值"="", "物理通道"=428, "逻辑通道"=140, "小数点"=1, "数值"=0.0, "修正因子"={"a"=0.0, "b"=1.0, "c"=0.0}, "原始值"=0.0, "逻辑名称"="Barometric Pressure(DP7)"}, {"展示名称"="25TR Indoor room dry bulb temp", "单位"="℃", "值"="", "物理通道"=429, "逻辑通道"=141, "小数点"=1, "数值"=0.0, "修正因子"={"a"=0.0, "b"=1.0, "c"=0.0}, "原始值"=0.0, "逻辑名称"="25TR Indoor room dry bulb temp"}, {"展示名称"="25TR Indoor room wet bulb temp", "单位"="℃", "值"="", "物理通道"=430, "逻辑通道"=142, "小数点"=1, "数值"=0.0, "修正因子"={"a"=0.0, "b"=1.0, "c"=0.0}, "原始值"=0.0, "逻辑名称"="25TR Indoor room wet bulb temp"}, {"展示名称"="50TR Indoor room dry bulb temp", "单位"="℃", "值"="", "物理通道"=431, "逻辑通道"=143, "小数点"=1, "数值"=0.0, "修正因子"={"a"=0.0, "b"=1.0, "c"=0.0}, "原始值"=0.0, "逻辑名称"="50TR Indoor room dry bulb temp"}, {"展示名称"="50TR Indoor room wet bulb temp", "单位"="℃", "值"="", "物理通道"=432, "逻辑通道"=144, "小数点"=1, "数值"=0.0, "修正因子"={"a"=0.0, "b"=1.0, "c"=0.0}, "原始值"=0.0, "逻辑名称"="50TR Indoor room wet bulb temp"}, {"展示名称"="50TR Outdoor room dry bulb temp1", "单位"="℃", "值"="", "物理通道"=433, "逻辑通道"=145, "小数点"=1, "数值"=0.0, "修正因子"={"a"=0.0, "b"=1.0, "c"=0.0}, "原始值"=0.0, "逻辑名称"="50TR Outdoor room dry bulb temp1"}, {"展示名称"="50TR Outdoor room wet bulb temp1", "单位"="℃", "值"="", "物理通道"=434, "逻辑通道"=146, "小数点"=1, "数值"=0.0, "修正因子"={"a"=0.0, "b"=1.0, "c"=0.0}, "原始值"=0.0, "逻辑名称"="50TR Outdoor room wet bulb temp1"}, {"展示名称"="50TR Outdoor room dry bulb temp2", "单位"="℃", "值"="", "物理通道"=435, "逻辑通道"=147, "小数点"=1, "数值"=0.0, "修正因子"={"a"=0.0, "b"=1.0, "c"=0.0}, "原始值"=0.0, "逻辑名称"="50TR Outdoor room dry bulb temp2"}, {"展示名称"="50TR Outdoor room wet bulb temp2", "单位"="℃", "值"="", "物理通道"=436, "逻辑通道"=148, "小数点"=1, "数值"=0.0, "修正因子"={"a"=0.0, "b"=1.0, "c"=0.0}, "原始值"=0.0, "逻辑名称"="50TR Outdoor room wet bulb temp2"}, {"展示名称"="25TR Small Chamber AC ESP", "单位"="Mpa", "值"="", "物理通道"=437, "逻辑通道"=149, "小数点"=1, "数值"=0.0, "修正因子"={"a"=0.0, "b"=1.0, "c"=0.0}, "原始值"=0.0, "逻辑名称"="25TR Small Chamber AC ESP"}, {"展示名称"="25TR Small Chamber B4 Nozzle SP", "单位"="Mpa", "值"="", "物理通道"=438, "逻辑通道"=150, "小数点"=1, "数值"=0.0, "修正因子"={"a"=0.0, "b"=1.0, "c"=0.0}, "原始值"=0.0, "逻辑名称"="25TR Small Chamber B4 Nozzle SP"}, {"展示名称"="25TR Big Chamber AC ESP", "单位"="Mpa", "值"="", "物理通道"=439, "逻辑通道"=151, "小数点"=1, "数值"=0.0, "修正因子"={"a"=0.0, "b"=1.0, "c"=0.0}, "原始值"=0.0, "逻辑名称"="25TR Big Chamber AC ESP"}, {"展示名称"="25TR Big Chamber B4 Nozzle SP", "单位"="Mpa", "值"="", "物理通道"=440, "逻辑通道"=152, "小数点"=1, "数值"=0.0, "修正因子"={"a"=0.0, "b"=1.0, "c"=0.0}, "原始值"=0.0, "逻辑名称"="25TR Big Chamber B4 Nozzle SP"}, {"展示名称"="50TR Small Chamber AC ESP", "单位"="Mpa", "值"="", "物理通道"=441, "逻辑通道"=153, "小数点"=1, "数值"=0.0, "修正因子"={"a"=0.0, "b"=1.0, "c"=0.0}, "原始值"=0.0, "逻辑名称"="50TR Small Chamber AC ESP"}, {"展示名称"="50TR Small Chamber B4 Nozzle SP", "单位"="Mpa", "值"="", "物理通道"=442, "逻辑通道"=154, "小数点"=1, "数值"=0.0, "修正因子"={"a"=0.0, "b"=1.0, "c"=0.0}, "原始值"=0.0, "逻辑名称"="50TR Small Chamber B4 Nozzle SP"}, {"展示名称"="50TR Big Chamber AC ESP", "单位"="Mpa", "值"="", "物理通道"=443, "逻辑通道"=155, "小数点"=1, "数值"=0.0, "修正因子"={"a"=0.0, "b"=1.0, "c"=0.0}, "原始值"=0.0, "逻辑名称"="50TR Big Chamber AC ESP"}, {"展示名称"="50TR Big Chamber B4 Nozzle SP", "单位"="Mpa", "值"="", "物理通道"=444, "逻辑通道"=156, "小数点"=1, "数值"=0.0, "修正因子"={"a"=0.0, "b"=1.0, "c"=0.0}, "原始值"=0.0, "逻辑名称"="50TR Big Chamber B4 Nozzle SP"}, {"展示名称"="FM1", "单位"="m3/h", "值"="", "物理通道"=445, "逻辑通道"=157, "小数点"=1, "数值"=0.0, "修正因子"={"a"=0.0, "b"=1.0, "c"=0.0}, "原始值"=0.0, "逻辑名称"="25TR Water System Water Flow Meter"}, {"展示名称"="FM2", "单位"="m3/h", "值"="", "物理通道"=446, "逻辑通道"=158, "小数点"=1, "数值"=0.0, "修正因子"={"a"=0.0, "b"=1.0, "c"=0.0}, "原始值"=0.0, "逻辑名称"="50TR Water System Water Flow Meter"}, {"展示名称"="50TR Small Chamber Nozzle Pressure Difference", "单位"="Mpa", "值"="", "物理通道"=448, "逻辑通道"=159, "小数点"=1, "数值"=0.0, "修正因子"={"a"=0.0, "b"=1.0, "c"=0.0}, "原始值"=0.0, "逻辑名称"="50TR Small Chamber Nozzle Pressure Difference"}, {"展示名称"="50TR Big Chamber Nozzle Pressure Difference", "单位"="Mpa", "值"="", "物理通道"=449, "逻辑通道"=160, "小数点"=1, "数值"=0.0, "修正因子"={"a"=0.0, "b"=1.0, "c"=0.0}, "原始值"=0.0, "逻辑名称"="50TR Big Chamber Nozzle Pressure Difference"}, {"展示名称"="25TR ID TC1", "单位"="℃", "值"="", "物理通道"=472, "逻辑通道"=161, "小数点"=1, "数值"=0.0, "修正因子"={"a"=0.0, "b"=1.0, "c"=0.0}, "原始值"=0.0, "逻辑名称"="TC1"}, {"展示名称"="25TR ID TC2", "单位"="℃", "值"="", "物理通道"=473, "逻辑通道"=162, "小数点"=1, "数值"=0.0, "修正因子"={"a"=0.0, "b"=1.0, "c"=0.0}, "原始值"=0.0, "逻辑名称"="TC2"}, {"展示名称"="25TR ID TC3", "单位"="℃", "值"="", "物理通道"=474, "逻辑通道"=163, "小数点"=1, "数值"=0.0, "修正因子"={"a"=0.0, "b"=1.0, "c"=0.0}, "原始值"=0.0, "逻辑名称"="TC3"}, {"展示名称"="25TR ID TC4", "单位"="℃", "值"="", "物理通道"=475, "逻辑通道"=164, "小数点"=1, "数值"=0.0, "修正因子"={"a"=0.0, "b"=1.0, "c"=0.0}, "原始值"=0.0, "逻辑名称"="TC4"}, {"展示名称"="25TR ID TC5", "单位"="℃", "值"="", "物理通道"=476, "逻辑通道"=165, "小数点"=1, "数值"=0.0, "修正因子"={"a"=0.0, "b"=1.0, "c"=0.0}, "原始值"=0.0, "逻辑名称"="TC5"}, {"展示名称"="25TR ID TC6", "单位"="℃", "值"="", "物理通道"=477, "逻辑通道"=166, "小数点"=1, "数值"=0.0, "修正因子"={"a"=0.0, "b"=1.0, "c"=0.0}, "原始值"=0.0, "逻辑名称"="TC6"}, {"展示名称"="25TR ID TC7", "单位"="℃", "值"="", "物理通道"=478, "逻辑通道"=167, "小数点"=2, "数值"=0.0, "修正因子"={"a"=0.0, "b"=1.0, "c"=0.0}, "原始值"=0.0, "逻辑名称"="TC7"}, {"展示名称"="25TR ID TC8", "单位"="℃", "值"="", "物理通道"=479, "逻辑通道"=168, "小数点"=1, "数值"=0.0, "修正因子"={"a"=0.0, "b"=1.0, "c"=0.0}, "原始值"=0.0, "逻辑名称"="TC8"}, {"展示名称"="25TR ID TC9", "单位"="℃", "值"="", "物理通道"=480, "逻辑通道"=169, "小数点"=1, "数值"=0.0, "修正因子"={"a"=0.0, "b"=1.0, "c"=0.0}, "原始值"=0.0, "逻辑名称"="TC9"}, {"展示名称"="25TR ID TC10", "单位"="℃", "值"="", "物理通道"=481, "逻辑通道"=170, "小数点"=1, "数值"=0.0, "修正因子"={"a"=0.0, "b"=1.0, "c"=0.0}, "原始值"=0.0, "逻辑名称"="TC10"}, {"展示名称"="25TR ID TC11", "单位"="℃", "值"="", "物理通道"=482, "逻辑通道"=171, "小数点"=2, "数值"=0.0, "修正因子"={"a"=0.0, "b"=1.0, "c"=0.0}, "原始值"=0.0, "逻辑名称"="TC11"}, {"展示名称"="25TR ID TC12", "单位"="℃", "值"="", "物理通道"=483, "逻辑通道"=172, "小数点"=1, "数值"=0.0, "修正因子"={"a"=0.0, "b"=1.0, "c"=0.0}, "原始值"=0.0, "逻辑名称"="TC12"}, {"展示名称"="25TR ID TC13", "单位"="℃", "值"="", "物理通道"=484, "逻辑通道"=173, "小数点"=1, "数值"=0.0, "修正因子"={"a"=0.0, "b"=1.0, "c"=0.0}, "原始值"=0.0, "逻辑名称"="TC13"}, {"展示名称"="25TR ID TC14", "单位"="℃", "值"="", "物理通道"=485, "逻辑通道"=174, "小数点"=1, "数值"=0.0, "修正因子"={"a"=0.0, "b"=1.0, "c"=0.0}, "原始值"=0.0, "逻辑名称"="TC14"}, {"展示名称"="25TR ID TC15", "单位"="℃", "值"="", "物理通道"=486, "逻辑通道"=175, "小数点"=2, "数值"=0.0, "修正因子"={"a"=0.0, "b"=1.0, "c"=0.0}, "原始值"=0.0, "逻辑名称"="TC15"}, {"展示名称"="25TR ID TC16", "单位"="℃", "值"="", "物理通道"=487, "逻辑通道"=176, "小数点"=1, "数值"=0.0, "修正因子"={"a"=0.0, "b"=1.0, "c"=0.0}, "原始值"=0.0, "逻辑名称"="TC16"}, {"展示名称"="25TR ID TC17", "单位"="℃", "值"="", "物理通道"=488, "逻辑通道"=177, "小数点"=1, "数值"=0.0, "修正因子"={"a"=0.0, "b"=1.0, "c"=0.0}, "原始值"=0.0, "逻辑名称"="TC17"}, {"展示名称"="25TR ID TC18", "单位"="℃", "值"="", "物理通道"=489, "逻辑通道"=178, "小数点"=1, "数值"=0.0, "修正因子"={"a"=0.0, "b"=1.0, "c"=0.0}, "原始值"=0.0, "逻辑名称"="TC18"}, {"展示名称"="25TR ID TC19", "单位"="℃", "值"="", "物理通道"=490, "逻辑通道"=179, "小数点"=2, "数值"=0.0, "修正因子"={"a"=0.0, "b"=1.0, "c"=0.0}, "原始值"=0.0, "逻辑名称"="TC19"}, {"展示名称"="25TR ID TC20", "单位"="℃", "值"="", "物理通道"=491, "逻辑通道"=180, "小数点"=1, "数值"=0.0, "修正因子"={"a"=0.0, "b"=1.0, "c"=0.0}, "原始值"=0.0, "逻辑名称"="TC20"}, {"展示名称"="50TR ID TC1", "单位"="℃", "值"="", "物理通道"=494, "逻辑通道"=181, "小数点"=1, "数值"=0.0, "修正因子"={"a"=0.0, "b"=1.0, "c"=0.0}, "原始值"=0.0, "逻辑名称"="TC1"}, {"展示名称"="50TR ID TC2", "单位"="℃", "值"="", "物理通道"=495, "逻辑通道"=182, "小数点"=1, "数值"=0.0, "修正因子"={"a"=0.0, "b"=1.0, "c"=0.0}, "原始值"=0.0, "逻辑名称"="TC2"}, {"展示名称"="50TR ID TC3", "单位"="℃", "值"="", "物理通道"=496, "逻辑通道"=183, "小数点"=2, "数值"=0.0, "修正因子"={"a"=0.0, "b"=1.0, "c"=0.0}, "原始值"=0.0, "逻辑名称"="TC3"}, {"展示名称"="50TR ID TC4", "单位"="℃", "值"="", "物理通道"=497, "逻辑通道"=184, "小数点"=1, "数值"=0.0, "修正因子"={"a"=0.0, "b"=1.0, "c"=0.0}, "原始值"=0.0, "逻辑名称"="TC4"}, {"展示名称"="50TR ID TC5", "单位"="℃", "值"="", "物理通道"=498, "逻辑通道"=185, "小数点"=2, "数值"=0.0, "修正因子"={"a"=0.0, "b"=1.0, "c"=0.0}, "原始值"=0.0, "逻辑名称"="TC5"}, {"展示名称"="50TR ID TC6", "单位"="℃", "值"="", "物理通道"=499, "逻辑通道"=186, "小数点"=1, "数值"=0.0, "修正因子"={"a"=0.0, "b"=1.0, "c"=0.0}, "原始值"=0.0, "逻辑名称"="TC6"}, {"展示名称"="50TR ID TC7", "单位"="℃", "值"="", "物理通道"=500, "逻辑通道"=187, "小数点"=1, "数值"=0.0, "修正因子"={"a"=0.0, "b"=1.0, "c"=0.0}, "原始值"=0.0, "逻辑名称"="TC7"}, {"展示名称"="50TR ID TC8", "单位"="℃", "值"="", "物理通道"=501, "逻辑通道"=188, "小数点"=1, "数值"=0.0, "修正因子"={"a"=0.0, "b"=1.0, "c"=0.0}, "原始值"=0.0, "逻辑名称"="TC8"}, {"展示名称"="50TR ID TC9", "单位"="℃", "值"="", "物理通道"=502, "逻辑通道"=189, "小数点"=2, "数值"=0.0, "修正因子"={"a"=0.0, "b"=1.0, "c"=0.0}, "原始值"=0.0, "逻辑名称"="TC9"}, {"展示名称"="50TR ID TC10", "单位"="℃", "值"="", "物理通道"=503, "逻辑通道"=190, "小数点"=1, "数值"=0.0, "修正因子"={"a"=0.0, "b"=1.0, "c"=0.0}, "原始值"=0.0, "逻辑名称"="TC10"}, {"展示名称"="50TR ID TC11", "单位"="℃", "值"="", "物理通道"=504, "逻辑通道"=191, "小数点"=1, "数值"=0.0, "修正因子"={"a"=0.0, "b"=1.0, "c"=0.0}, "原始值"=0.0, "逻辑名称"="TC11"}, {"展示名称"="50TR ID TC12", "单位"="℃", "值"="", "物理通道"=505, "逻辑通道"=192, "小数点"=1, "数值"=0.0, "修正因子"={"a"=0.0, "b"=1.0, "c"=0.0}, "原始值"=0.0, "逻辑名称"="TC12"}, {"展示名称"="50TR ID TC13", "单位"="℃", "值"="", "物理通道"=506, "逻辑通道"=193, "小数点"=2, "数值"=0.0, "修正因子"={"a"=0.0, "b"=1.0, "c"=0.0}, "原始值"=0.0, "逻辑名称"="TC13"}, {"展示名称"="50TR ID TC14", "单位"="℃", "值"="", "物理通道"=507, "逻辑通道"=194, "小数点"=1, "数值"=0.0, "修正因子"={"a"=0.0, "b"=1.0, "c"=0.0}, "原始值"=0.0, "逻辑名称"="TC14"}, {"展示名称"="50TR ID TC15", "单位"="℃", "值"="", "物理通道"=508, "逻辑通道"=195, "小数点"=1, "数值"=0.0, "修正因子"={"a"=0.0, "b"=1.0, "c"=0.0}, "原始值"=0.0, "逻辑名称"="TC15"}, {"展示名称"="50TR ID TC16", "单位"="℃", "值"="", "物理通道"=509, "逻辑通道"=196, "小数点"=1, "数值"=0.0, "修正因子"={"a"=0.0, "b"=1.0, "c"=0.0}, "原始值"=0.0, "逻辑名称"="TC16"}, {"展示名称"="50TR ID TC17", "单位"="℃", "值"="", "物理通道"=510, "逻辑通道"=197, "小数点"=2, "数值"=0.0, "修正因子"={"a"=0.0, "b"=1.0, "c"=0.0}, "原始值"=0.0, "逻辑名称"="TC17"}, {"展示名称"="50TR ID TC18", "单位"="℃", "值"="", "物理通道"=511, "逻辑通道"=198, "小数点"=1, "数值"=0.0, "修正因子"={"a"=0.0, "b"=1.0, "c"=0.0}, "原始值"=0.0, "逻辑名称"="TC18"}, {"展示名称"="50TR ID TC19", "单位"="℃", "值"="", "物理通道"=512, "逻辑通道"=199, "小数点"=1, "数值"=0.0, "修正因子"={"a"=0.0, "b"=1.0, "c"=0.0}, "原始值"=0.0, "逻辑名称"="TC19"}, {"展示名称"="50TR ID TC20", "单位"="℃", "值"="", "物理通道"=513, "逻辑通道"=200, "小数点"=1, "数值"=0.0, "修正因子"={"a"=0.0, "b"=1.0, "c"=0.0}, "原始值"=0.0, "逻辑名称"="TC20"}, {"展示名称"="50TR OD TC1", "单位"="℃", "值"="", "物理通道"=516, "逻辑通道"=201, "小数点"=2, "数值"=0.0, "修正因子"={"a"=0.0, "b"=1.0, "c"=0.0}, "原始值"=0.0, "逻辑名称"="TC1"}, {"展示名称"="50TR OD TC2", "单位"="℃", "值"="", "物理通道"=517, "逻辑通道"=202, "小数点"=2, "数值"=0.0, "修正因子"={"a"=0.0, "b"=1.0, "c"=0.0}, "原始值"=0.0, "逻辑名称"="TC2"}, {"展示名称"="50TR OD TC3", "单位"="℃", "值"="", "物理通道"=518, "逻辑通道"=203, "小数点"=1, "数值"=0.0, "修正因子"={"a"=0.0, "b"=1.0, "c"=0.0}, "原始值"=0.0, "逻辑名称"="TC3"}, {"展示名称"="50TR OD TC4", "单位"="℃", "值"="", "物理通道"=519, "逻辑通道"=204, "小数点"=2, "数值"=0.0, "修正因子"={"a"=0.0, "b"=1.0, "c"=0.0}, "原始值"=0.0, "逻辑名称"="TC4"}, {"展示名称"="50TR OD TC5", "单位"="℃", "值"="", "物理通道"=520, "逻辑通道"=205, "小数点"=2, "数值"=0.0, "修正因子"={"a"=0.0, "b"=1.0, "c"=0.0}, "原始值"=0.0, "逻辑名称"="TC5"}, {"展示名称"="50TR OD TC6", "单位"="℃", "值"="", "物理通道"=521, "逻辑通道"=206, "小数点"=2, "数值"=0.0, "修正因子"={"a"=0.0, "b"=1.0, "c"=0.0}, "原始值"=0.0, "逻辑名称"="TC6"}, {"展示名称"="50TR OD TC7", "单位"="℃", "值"="", "物理通道"=522, "逻辑通道"=207, "小数点"=2, "数值"=0.0, "修正因子"={"a"=0.0, "b"=1.0, "c"=0.0}, "原始值"=0.0, "逻辑名称"="TC7"}, {"展示名称"="50TR OD TC8", "单位"="℃", "值"="", "物理通道"=523, "逻辑通道"=208, "小数点"=2, "数值"=0.0, "修正因子"={"a"=0.0, "b"=1.0, "c"=0.0}, "原始值"=0.0, "逻辑名称"="TC8"}, {"展示名称"="50TR OD TC9", "单位"="℃", "值"="", "物理通道"=524, "逻辑通道"=209, "小数点"=2, "数值"=0.0, "修正因子"={"a"=0.0, "b"=1.0, "c"=0.0}, "原始值"=0.0, "逻辑名称"="TC9"}, {"展示名称"="50TR OD TC10", "单位"="℃", "值"="", "物理通道"=525, "逻辑通道"=210, "小数点"=1, "数值"=0.0, "修正因子"={"a"=0.0, "b"=1.0, "c"=0.0}, "原始值"=0.0, "逻辑名称"="TC10"}, {"展示名称"="50TR OD TC11", "单位"="℃", "值"="", "物理通道"=526, "逻辑通道"=211, "小数点"=1, "数值"=0.0, "修正因子"={"a"=0.0, "b"=1.0, "c"=0.0}, "原始值"=0.0, "逻辑名称"="TC11"}, {"展示名称"="50TR OD TC12", "单位"="℃", "值"="", "物理通道"=527, "逻辑通道"=212, "小数点"=2, "数值"=0.0, "修正因子"={"a"=0.0, "b"=1.0, "c"=0.0}, "原始值"=0.0, "逻辑名称"="TC12"}, {"展示名称"="50TR OD TC13", "单位"="℃", "值"="", "物理通道"=528, "逻辑通道"=213, "小数点"=2, "数值"=0.0, "修正因子"={"a"=0.0, "b"=1.0, "c"=0.0}, "原始值"=0.0, "逻辑名称"="TC13"}, {"展示名称"="50TR OD TC14", "单位"="℃", "值"="", "物理通道"=529, "逻辑通道"=214, "小数点"=2, "数值"=0.0, "修正因子"={"a"=0.0, "b"=1.0, "c"=0.0}, "原始值"=0.0, "逻辑名称"="TC14"}, {"展示名称"="50TR OD TC15", "单位"="℃", "值"="", "物理通道"=530, "逻辑通道"=215, "小数点"=2, "数值"=0.0, "修正因子"={"a"=0.0, "b"=1.0, "c"=0.0}, "原始值"=0.0, "逻辑名称"="TC15"}, {"展示名称"="50TR OD TC16", "单位"="℃", "值"="", "物理通道"=531, "逻辑通道"=216, "小数点"=2, "数值"=0.0, "修正因子"={"a"=0.0, "b"=1.0, "c"=0.0}, "原始值"=0.0, "逻辑名称"="TC16"}, {"展示名称"="50TR OD TC17", "单位"="℃", "值"="", "物理通道"=532, "逻辑通道"=217, "小数点"=2, "数值"=0.0, "修正因子"={"a"=0.0, "b"=1.0, "c"=0.0}, "原始值"=0.0, "逻辑名称"="TC17"}, {"展示名称"="50TR OD TC18", "单位"="℃", "值"="", "物理通道"=533, "逻辑通道"=218, "小数点"=1, "数值"=0.0, "修正因子"={"a"=0.0, "b"=1.0, "c"=0.0}, "原始值"=0.0, "逻辑名称"="TC18"}, {"展示名称"="50TR OD TC19", "单位"="℃", "值"="", "物理通道"=534, "逻辑通道"=219, "小数点"=1, "数值"=0.0, "修正因子"={"a"=0.0, "b"=1.0, "c"=0.0}, "原始值"=0.0, "逻辑名称"="TC19"}, {"展示名称"="50TR OD TC20", "单位"="℃", "值"="", "物理通道"=535, "逻辑通道"=220, "小数点"=1, "数值"=0.0, "修正因子"={"a"=0.0, "b"=1.0, "c"=0.0}, "原始值"=0.0, "逻辑名称"="TC20"}]
  in  "TestID":string
  in  "工况设置":T2={"Test Type"=0, "FM"=1.0, "Eva Power"=1.0, "Comp Power"=1.0, "Cond Power"=1.0, "Dis Pre"=["SP1", "SP2", "SP3", "Average SP", "", "", "", "", "", ""], "Suc Pre"=["SP5", "SP6", "SP7", "SP8", "", "", "", "", "", ""], "Dis Tem"=["TC117", "TC118", "TC119", "TC120", "", "", "", "", "", ""], "Suc Tem"=["TC121", "TC122", "TC123", "TC124", "", "", "", "", "", ""], "Liquid Tem"=["TC125", "TC126", "TC127", "TC128", "", "", "", "", "", ""], "Oil Pre"=["SP1", "SP2", "SP3", "SP4", "", "", "", "", "", ""], "Leaving Air Temp"=["TC117", "TC118", "TC119", "TC120", "", "", "", "", "", ""], "Liquid Pre"=["SP9", "SP10", "SP11", "SP12", "", "", "", "", "", ""], "Tested Unit Outlet Dry Temp"=[], "Compressor Temp"=["25TR ID TC11", "25TR ID TC12", "25TR ID TC13", "25TR ID TC14", "25TR ID TC15", "25TR ID TC16", "25TR ID TC17", "25TR ID TC18", "25TR ID TC19", "25TR ID TC20"], "Evap.Leaving Temp"=[], "Evap.Entering Temp"=[], "25TR SP Choose1"=["", "", "", "", "", "", "", "", "", ""], "25TR SP Choose2"=["", "", "", "", "", "", "", "", "", ""], "25TR Temp Choose2"=["25TR ID TC11", "25TR ID TC12", "25TR ID TC13", "25TR ID TC14", "25TR ID TC15", "25TR ID TC16", "25TR ID TC17", "25TR ID TC18", "25TR ID TC19", "25TR ID TC20"], "25TR Temp Choose"=["25TR ID TC1", "25TR ID TC2", "25TR ID TC3", "25TR ID TC4", "25TR ID TC5", "25TR ID TC6", "25TR ID TC7", "25TR ID TC8", "25TR ID TC9", "25TR ID TC10"], "Ref Type"="", "Left Chamber Selected"=0, "OD Dry Temp"=["PT5", "PT5", "", "", "", "", "", "", "", "", "", ""], "OD Wet Temp"=["PT6", "PT8", "", "", "", "", "", "", "", "", "", ""], "OD RH"=["RH1", "RH2", "", "", "", "", "", "", "", "", "", ""]} {"Left Chamber Selected" items=["None", "25TR Small", "25TR Big"]; "Test Type" items=["Cooling", "Heating"]}
  out "Test Type":i16
  out "Default":bool
  out "Test Kind":i16
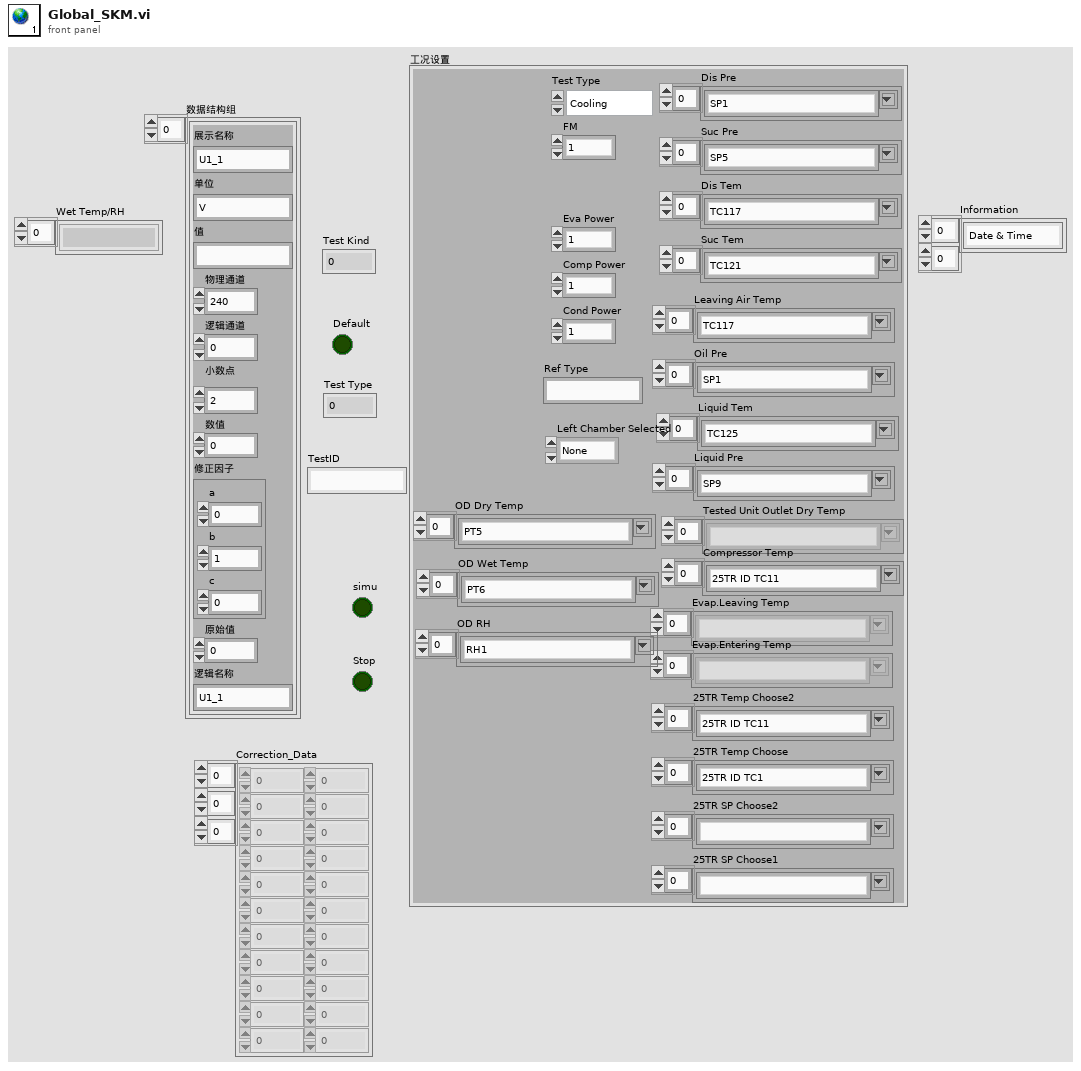
[diagram p1: front panel]
types:
  T1 = typedef "data structure.ctl" = cluster{"展示名称":string, "单位":string, "值":string, "物理通道":i32, "逻辑通道":i32, "小数点":i16, "数值":dbl, "修正因子":cluster{"a":dbl, "b":dbl, "c":dbl}, "原始值":sgl, "逻辑名称":string}
  T2 = typedef "Working condition setting_SKM.ctl" = cluster{"Test Type":u16, "FM":dbl, "Eva Power":dbl, "Comp Power":dbl, "Cond Power":dbl, "Dis Pre":string[], "Suc Pre":string[], "Dis Tem":string[], "Suc Tem":string[], "Liquid Tem":string[], "Oil Pre":string[], "Leaving Air Temp":string[], "Liquid Pre":string[], "Tested Unit Outlet Dry Temp":string[], "Compressor Temp":string[], "Evap.Leaving Temp":string[], "Evap.Entering Temp":string[], "25TR SP Choose1":string[], "25TR SP Choose2":string[], "25TR Temp Choose2":string[], "25TR Temp Choose":string[], "Ref Type":string, "Left Chamber Selected":u16, "OD Dry Temp":string[], "OD Wet Temp":string[], "OD RH":string[]}
diagram:
